vi "DiffDrivePoseEst2_InterpRecord_Interp.vi"(6 "Extra":variant, 9 "Time Fraction":dbl, 10 "End Input 2":variant, 11 "Input 1":variant) -> (3 "Interp Output":variant)   [LabVIEW 2019, in "Trajectory_Library.lvlib"]
doc: "Return the interpolated record. This object is assumed to be the starting position, or lower bound.\n\nInputs:\n - Input 1 -- The lower bound data cluster\n - end Input 2 -- The upper bound, or end, data cluster\n - time frac -- How far between the lower and upper bound we are. This should be bounded in [0, 1].\n - extra -- variant -- extra data needed for the calculation.\n\nReturns:\n - The interpolated cluster value."
uses:
  Trajectory_Library.lvlib
  TypeDef/DIFF_DRIVE_KINEMATICS.ctl
  Rotation2d_Plus.vi
  MathUtil_Clamp.vi
  Rotation2d_Times.vi
  Rotation2d_UnaryMinus.vi
  Rotation2d_RotateBy.vi
  Twist2d_Create.vi
  Rotation2d_CreateAngle.vi
  Rotation2d_CreateXY.vi
  Util_CalcDist.vi
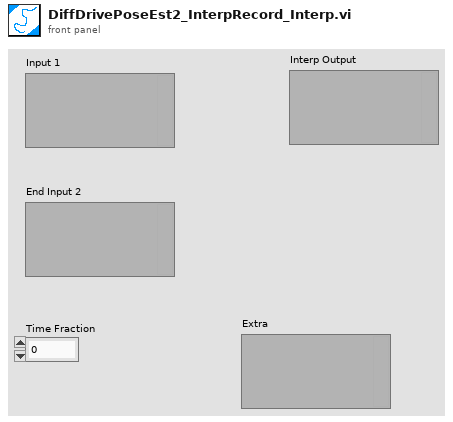
[diagram p1: front panel]
types:
  T1 = typedef "Trajectory_Library.lvlib/DIFF_DRIVE_POSE_EST2_INTERP_RECORD.ctl" = cluster{"PoseMeters":T2, "GyroAngle":T4, "LeftMeters":dbl, "RightMeters":dbl}
  T2 = typedef "Trajectory_Library.lvlib/POSE2D.ctl" = cluster{"TRANSLATION":T3, "ROTATION":T4}
  T3 = typedef "Trajectory_Library.lvlib/TRANSLATION2D.ctl" = cluster{"X":dbl, "Y":dbl}
  T4 = typedef "Trajectory_Library.lvlib/ROTATION2D.ctl" = cluster{"VALUE":dbl, "COS":dbl, "SIN":dbl}
  T5 = typedef "Trajectory_Library.lvlib/DIFF_DRIVE_KINEMATICS.ctl" = cluster{"TrackWidth_Meters":dbl}
  T6 = typedef "Trajectory_Library.lvlib/TWIST2D.ctl" = cluster{"dX":dbl, "dY":dbl, "dTHETA":dbl}
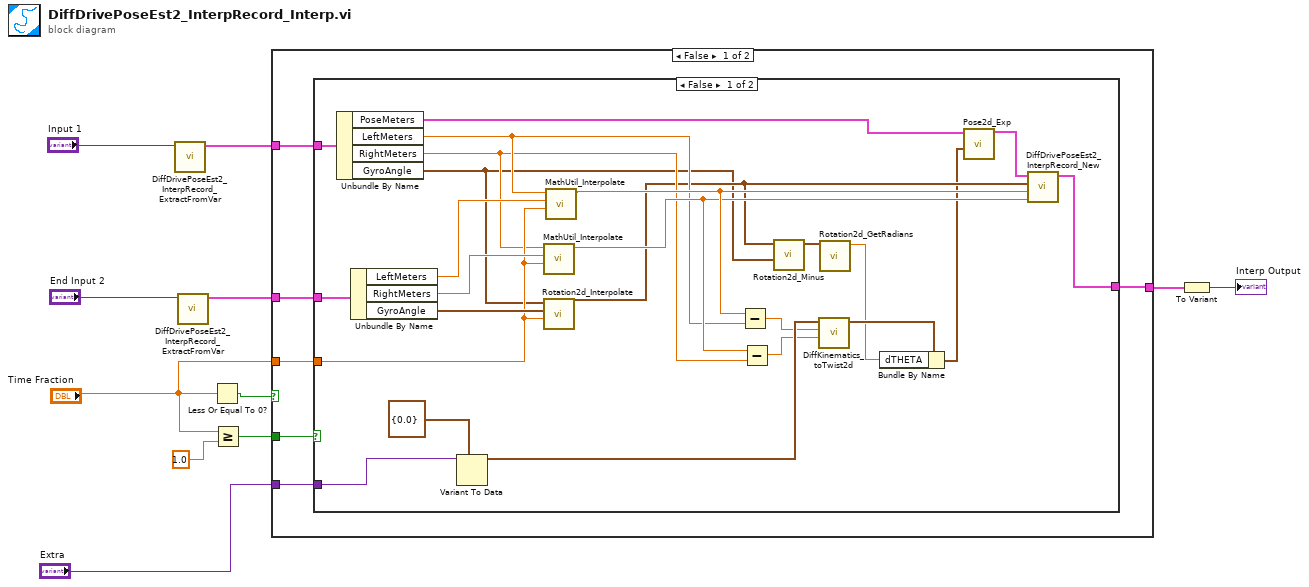
[diagram p0: block diagram]
diagram:
  n1 = call "DiffDrivePoseEst2_InterpRecord_ExtractFromVar.vi"("OutputVariant"="Input 1") -> ("out InterpRecord"=w3:T1)  [unwired: 9 in, 1 out]
  n2 = call "DiffDrivePoseEst2_InterpRecord_ExtractFromVar.vi"("OutputVariant"="End Input 2") -> ("out InterpRecord"=w1:T1)  [unwired: 9 in, 1 out]
  n3 = Less Or Equal To 0?(x="Time Fraction") -> (x <= 0?=w11:bool)
  n4 = Greater Or Equal?(x="Time Fraction", y=1.0) -> (x >= y?=w7:bool)
  n5 = case shown="False" w11 {
    tunnel: [w16 w43] -> w9
    tunnel: w3 -> [w14 w43]
    tunnel: w7 -> [w17 _]
    tunnel: w1 -> [w15 _]
    tunnel: "Time Fraction" -> [w13 _]
    tunnel: "Extra" -> [w12 _]
    frame False {
      n6 = case shown="False" w17 {
        tunnel: [w18 w42] -> w16
        tunnel: w15 -> [w40 w42]
        tunnel: w14 -> [w41 _]
        tunnel: w13 -> [w36 _]
        tunnel: w12 -> [w35 _]
        frame False {
          n7 = Unbundle By Name(w41) -> ("PoseMeters"=w21:T2, "LeftMeters"=w31:dbl, "RightMeters"=w30:dbl, "GyroAngle"=w24:T4)
          n8 = Unbundle By Name(w40) -> ("LeftMeters"=w39:dbl, "RightMeters"=w38:dbl, "GyroAngle"=w37:T4)
          n9 = Variant To Data(type=T5 {"TrackWidth_Meters"=0.0} ("DIFF_DRIVE_KINEMATICS"), Variant=w35) -> (data=w29:T5)  [unwired: 1 in, 1 out]
          n10 = call "MathUtil_Interpolate.vi"("T"=w36, "EndValue"=w38, "StartValue"=w30) -> ("InterpolatedValue"=w32:dbl)  [unwired: 8 in]
          n11 = call "Rotation2d_Interpolate.vi"("T"=w36, "EncValue ROTATION"=w37, "in ROTATION"=w24) -> ("Interpolated ROTATION"=w25:T4)  [unwired: 8 in]
          n12 = call "MathUtil_Interpolate.vi"("T"=w36, "EndValue"=w39, "StartValue"=w31) -> ("InterpolatedValue"=w33:dbl)  [unwired: 8 in]
          n13 = Subtract(x=w33, y=w31) -> (x-y=w28:dbl)
          n14 = Subtract(x=w32, y=w30) -> (x-y=w27:dbl)
          n15 = call "Rotation2d_Minus.vi"("other ROTATION"=w24, "in ROTATION"=w25) -> ("out ROTATION"=w23:T4)  [unwired: 9 in]
          n16 = call "DiffKinematics_toTwist2d.vi"("Right Distance M"=w27, "Left Distance M"=w28, "DIFF_DRIVE_KINEMATICS"=w29) -> ("Twist2d"=w26:T6)  [unwired: 8 in]
          n17 = call "Rotation2d_GetRadians.vi"("in ROTATION"=w23) -> ("AngleRadians"=w22:dbl)  [unwired: 10 in]
          n18 = Bundle By Name(cluster=w26, "dTHETA"=w22) -> (w19:T6)
          n19 = call "Pose2d_Exp.vi"("TWIST"=w19, "POSE"=w21) -> ("UpdatedPose"=w20:T2)  [unwired: 9 in]
          n20 = call "DiffDrivePoseEst2_InterpRecord_New.vi"("RightDistance"=w32, "LeftDistance"=w33, "GyroAngle"=w25, "M_POSE_Meters"=w20) -> ("DIFF_DRIVE_POSE_EST2_INTERP_RECORD"=w18:T1)  [unwired: 7 in]
        }
        frame True {
        }
      }
    }
    frame True {
    }
  }
  n21 = To Variant(anything=w9) -> (Variant=→"Interp Output":variant)
